vi "ServoController.vi"   [LabVIEW 2026]
uses:
  <vilib>/DAQmx/write.llb/DAQmx Write (Counter Time 1Chan 1Samp).vi
  <vilib>/DAQmx/create/channels.llb/DAQmx Create Channel (CO-Pulse Generation-Time).vi
  <vilib>/DAQmx/configure/timing.llb/DAQmx Timing (Implicit).vi
  StateMachine/Globals.vi
  <vilib>/DAQmx/miscellaneous.llb/DAQmx Fill In Error Info.vi
types:
  T1 = typedef "ServoCommand.ctl" = enum16{"colour 1", "Colour2", "Colour3", "Reject"}
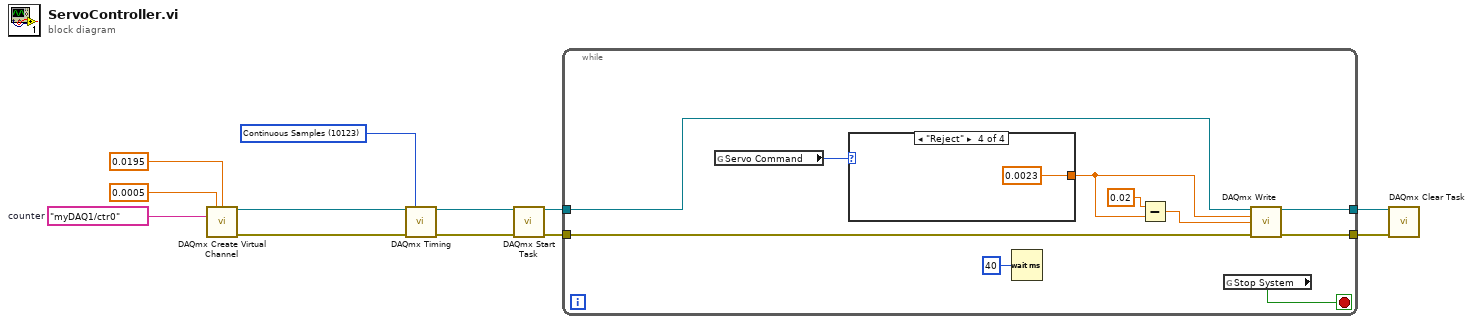
[diagram p0: block diagram]
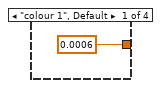
[diagram p2: hidden frame]
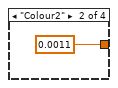
[diagram p3: hidden frame]
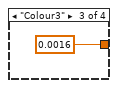
[diagram p4: hidden frame]
diagram:
  w3 = 10123 items=["Finite Samples"=10178, "Continuous Samples"=10123, "Hardware Timed Single Point"=12522] ("sample mode")
  w12 = tag "myDAQ1/ctr0"  # counter
  n1 = call-poly <vilib>:"DAQmx Create Virtual Channel.vi"("high time"=0.0005, "low time"=0.0195, "counter"=w12) -> ("task out"=w5:refnum<k21>, "error out"=w4:errorcluster)  [unwired: 11 in]
  n2 = call-poly <vilib>:"DAQmx Timing.vi"("task/channels in"=w5, "sample mode"=w3, "error in"=w4) -> ("task out"=w2:refnum<k21>, "error out"=w1:errorcluster)  [unwired: 11 in]
  n3 = call <vilib>:"DAQmx Start Task.vi"("task/channels in"=w2, "error in"=w1) -> ("task out"=w11:refnum<k21>, "error out"=w10:errorcluster)  [unwired: 12 in]
  n4 = while {
    tunnel: w11 -> [w20]
    tunnel: w10 -> [w19]
    tunnel: [w18] -> w9
    tunnel: [w17] -> w8
    stop <- w22 stop-if-true
    n5 = global read "Globals.vi" "Servo Command"() -> (w14:T1)
    n6 = case shown="\"Reject\"" w14 {
      tunnel: [0.0006 0.0011 0.0016 0.0023] -> w13
      frame "colour 1", Default {
      }
      frame "Colour2" {
      }
      frame "Colour3" {
      }
      frame "Reject" {
      }
    }
    n7 = Wait (ms)(milliseconds to wait=u32 40) -> ()  [unwired: 1 out]
    n8 = Subtract(x=0.02, y=w13) -> (x-y=w16:dbl)
    n9 = global read "Globals.vi" "Stop System"() -> (w22:bool)
    n10 = call-poly <vilib>:"DAQmx Write.vi"("task/channels in"=w20, "high time"=w13, "low time"=w16, "error in"=w19) -> ("task out"=w18:refnum<k21>, "error out"=w17:errorcluster)  [unwired: 9 in, 1 out]
  }
  n11 = call <vilib>:"DAQmx Clear Task.vi"("task in"=w9, "error in"=w8) -> ()  [unwired: 13 in, 1 out]
